vi "MotionProfileControlsInit.vi"() -> (0 "MotionPlanningNotifiers":T1)   [LabVIEW 2017]
uses:
  TypeDefs/RobotComponents/MotionPlanningNotifiers.ctl
  Autonomous/PathPlannerSupport/TypeDefs/DrivePlanRequest.ctl
  Autonomous/TypeDef/AutoWaypointType.ctl
  Pathfinder/Pathfinder-LabVIEW/Pathfinder-Lib/VIs/Waypoint.ctl
  Autonomous/PathPlannerSupport/TypeDefs/DrivePlanResponse.ctl
  Pathfinder/Pathfinder-LabVIEW/Pathfinder-Lib/VIs/Segment.ctl
  Implements/Arm/TypeDefs/ArmPlanRequest.ctl
  Implements/Arm/TypeDefs/ArmTargetPosition.ctl
  Implements/Arm/TypeDefs/ArmPlanResponse.ctl
  General/MotionProfiling/TypeDefs/TrajectoryPoint.ctl
  <vilib>/Rock Robotics/WPI/ThirdParty/Phoenix-LabVIEW/Motor Controller/Controls/CTRE_Phoenix_MotorControl_TrajectoryPointTimeDur.ctl
  General/MotionProfiling/TypeDefs/ArmMotionProfileControl.ctl
  General/MotionProfiling/TypeDefs/DriveMotionProfileControl.ctl
  MotionProfileControlData.vi
  Pathfinder/Pathfinder-LabVIEW/Pathfinder-Lib/Pathfinder.lvlib
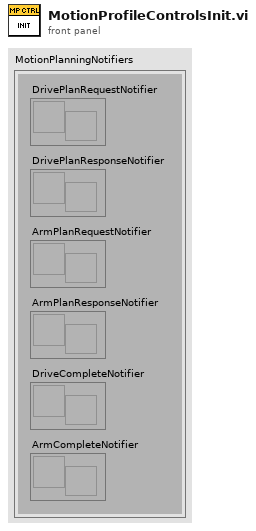
[diagram p1: front panel]
types:
  T1 = typedef "MotionPlanningNotifiers.ctl" = cluster{"DrivePlanRequestNotifier":refnum<notifier>, "DrivePlanResponseNotifier":refnum<notifier>, "ArmPlanRequestNotifier":refnum<notifier>, "ArmPlanResponseNotifier":refnum<notifier>, "DriveCompleteNotifier":refnum<notifier>, "ArmCompleteNotifier":refnum<notifier>}
  T2 = typedef "Pathfinder.lvlib/Segment.ctl" = cluster{"dt":dbl, "x":dbl, "y":dbl, "position":dbl, "velocity":dbl, "acceleration":dbl, "jerk":dbl, "heading":dbl}
  T3 = typedef "ArmPlanResponse.ctl" = cluster{"RotateTrajectory":T4[], "ExtendTrajectory":T4[], "PlanTime (ms)":u32, "Execute":bool}
  T4 = typedef "TrajectoryPoint.ctl" = cluster{"Position ":dbl, "Velocity ":dbl, "Time (ms)":T5, "Last Point":bool}
  T5 = typedef "CTRE_Phoenix_MotorControl_TrajectoryPointTimeDur.ctl" = i32
  T6 = typedef "ArmPlanRequest.ctl" = cluster{"Destination":T7, "Preview":bool}
  T7 = typedef "ArmTargetPosition.ctl" = enum16{"Hold", "Grab", "Switch", "Scale Low", "Scale High"}
  T8 = typedef "DrivePlanResponse.ctl" = cluster{"LeftDriveTrajectory":T2[], "RightDriveTrajectory":T2[], "PlanTime (ms)":u32, "Execute":bool}
  T9 = typedef "DrivePlanRequest.ctl" = cluster{"Plan Type":T10, "Waypoints":T11[], "Preview":bool}
  T10 = typedef "AutoWaypointType.ctl" = enum16{"Pathfinder Endpoint", "Pathfinder Waypoint", "Zero-Radius Turn Endpoint", "Stationary", "Vision Assist Endpoint"}
  T11 = typedef "Pathfinder.lvlib/Waypoint.ctl" = cluster{"x":dbl, "y":dbl, "angle":dbl}
  T12 = typedef "DriveMotionProfileControl.ctl" = cluster{"ControlMutex":T13, "Trajectory Points":T2[], "CurrentIndex":u32}
  T13 = typedef "Semaphore RefNum" = refnum<k1>
  T14 = typedef "ArmMotionProfileControl.ctl" = cluster{"ControlMutex":T13, "Trajectory Points":T4[], "CurrentIndex":u32}
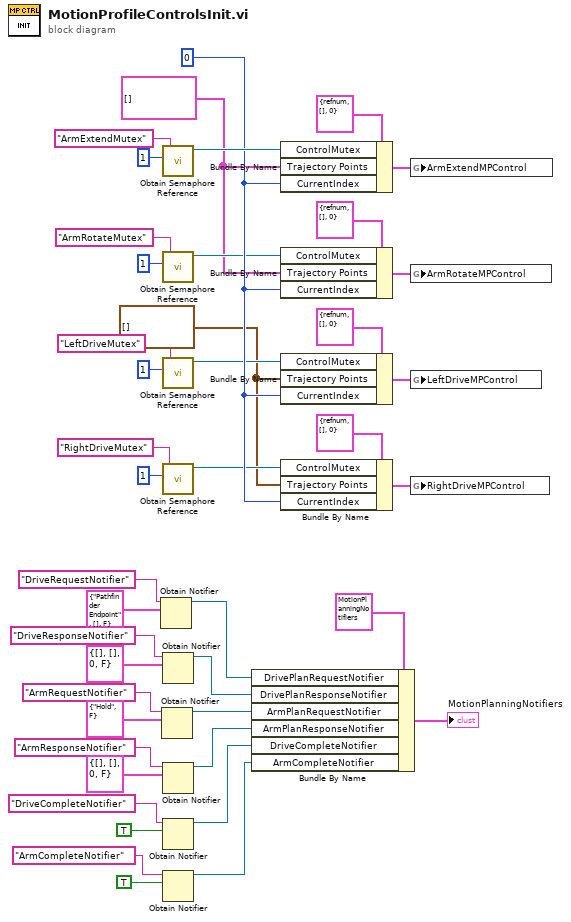
[diagram p0: block diagram]
diagram:
  w15 = T2[] [] ("Trajectory Points")
  w30 = u32 0 ("ArmExtendMPControl.CurrentIndex")
  w26 = T4[] [] ("ArmExtendMPControl.Trajectory Points")
  n1 = Obtain Notifier(name (unnamed)="DriveRequestNotifier", notification data type=T9 {"Plan Type"=enum."Pathfinder Endpoint", "Waypoints"=[], "Preview"=FALSE} ("DrivePlanRequest")) -> (notifier out=w19:refnum<notifier>)  [unwired: 2 in, 2 out]
  n2 = Obtain Notifier(name (unnamed)="ArmRequestNotifier", notification data type=T6 {"Destination"=enum."Hold", "Preview"=FALSE} ("ArmPlanRequest")) -> (notifier out=w17:refnum<notifier>)  [unwired: 2 in, 2 out]
  n3 = call <vilib>:"Obtain Semaphore Reference.vi"("size (1)"=1, "name (unnamed)"="ArmExtendMutex") -> ("semaphore"=w43:T13)  [unwired: 3 in, 2 out]
  n4 = call <vilib>:"Obtain Semaphore Reference.vi"("size (1)"=1, "name (unnamed)"="ArmRotateMutex") -> ("semaphore"=w29:T13)  [unwired: 3 in, 2 out]
  n5 = call <vilib>:"Obtain Semaphore Reference.vi"("size (1)"=1, "name (unnamed)"="LeftDriveMutex") -> ("semaphore"=w28:T13)  [unwired: 3 in, 2 out]
  n6 = call <vilib>:"Obtain Semaphore Reference.vi"("size (1)"=1, "name (unnamed)"="RightDriveMutex") -> ("semaphore"=w27:T13)  [unwired: 3 in, 2 out]
  n7 = Obtain Notifier(name (unnamed)="DriveResponseNotifier", notification data type=T8 {"LeftDriveTrajectory"=[], "RightDriveTrajectory"=[], "PlanTime (ms)"=0, "Execute"=FALSE} ("DrivePlanResponse")) -> (notifier out=w18:refnum<notifier>)  [unwired: 2 in, 2 out]
  n8 = Obtain Notifier(name (unnamed)="ArmResponseNotifier", notification data type=T3 {"RotateTrajectory"=[], "ExtendTrajectory"=[], "PlanTime (ms)"=0, "Execute"=FALSE} ("ArmPlanResponse")) -> (notifier out=w16:refnum<notifier>)  [unwired: 2 in, 2 out]
  n9 = Obtain Notifier(name (unnamed)="DriveCompleteNotifier", notification data type=TRUE) -> (notifier out=w2:refnum<notifier>)  [unwired: 2 in, 2 out]
  n10 = Obtain Notifier(name (unnamed)="ArmCompleteNotifier", notification data type=TRUE) -> (notifier out=w1:refnum<notifier>)  [unwired: 2 in, 2 out]
  n11 = Bundle By Name(cluster=T1 {"DrivePlanRequestNotifier"=refnum, "DrivePlanResponseNotifier"=refnum, "ArmPlanRequestNotifier"=refnum, "ArmPlanResponseNotifier"=refnum, "DriveCompleteNotifier"=refnum, "ArmCompleteNotifier"=refnum} ("MotionPlanningNotifiers"), "DrivePlanRequestNotifier"=w19, "DrivePlanResponseNotifier"=w18, "ArmPlanRequestNotifier"=w17, "ArmPlanResponseNotifier"=w16, "DriveCompleteNotifier"=w2, "ArmCompleteNotifier"=w1) -> (→"MotionPlanningNotifiers":T1)
  n12 = Bundle By Name(cluster=T14 {"ControlMutex"=refnum, "Trajectory Points"=[], "CurrentIndex"=0} ("MotionProfileControl"), "ControlMutex"=w43, "Trajectory Points"=w26, "CurrentIndex"=w30) -> (w38:T14)
  n13 = Bundle By Name(cluster=T14 {"ControlMutex"=refnum, "Trajectory Points"=[], "CurrentIndex"=0} ("MotionProfileControl"), "ControlMutex"=w29, "Trajectory Points"=w26, "CurrentIndex"=w30) -> (w35:T14)
  n14 = Bundle By Name(cluster=T12 {"ControlMutex"=refnum, "Trajectory Points"=[], "CurrentIndex"=0} ("MotionProfileControl"), "ControlMutex"=w28, "Trajectory Points"=w15, "CurrentIndex"=w30) -> (w34:T12)
  n15 = Bundle By Name(cluster=T12 {"ControlMutex"=refnum, "Trajectory Points"=[], "CurrentIndex"=0} ("MotionProfileControl"), "ControlMutex"=w27, "Trajectory Points"=w15, "CurrentIndex"=w30) -> (w31:T12)
  n16 = global write "MotionProfileControlData.vi" "ArmExtendMPControl"(w38) -> ()
  n17 = global write "MotionProfileControlData.vi" "ArmRotateMPControl"(w35) -> ()
  n18 = global write "MotionProfileControlData.vi" "LeftDriveMPControl"(w34) -> ()
  n19 = global write "MotionProfileControlData.vi" "RightDriveMPControl"(w31) -> ()
